vi "Teardown.vi"(8 "error in (no error)":errorcluster, 11 "LUnit Process Test In":refnum<class "Process Test.lvclass">) -> (0 "error out":errorcluster, 3 "LUnit Process Test Out":refnum<class "Process Test.lvclass">)   [LabVIEW 2020, in "Process Test.lvclass"]
uses:
  Process Test.lvclass
  Process Test.lvclass/Process Test.ctl
  C:/Git/astemes-triarc-framework/source/Framework Test Suite/Base Class Test/Base Test.lvclass
  C:/Program Files (x86)/National Instruments/LabVIEW 2020/vi.lib/Astemes/LUnit/Test Case.lvclass
  C:/Git/astemes-triarc-framework/source/Framework Test Suite/Process Test/Process Test.lvclass
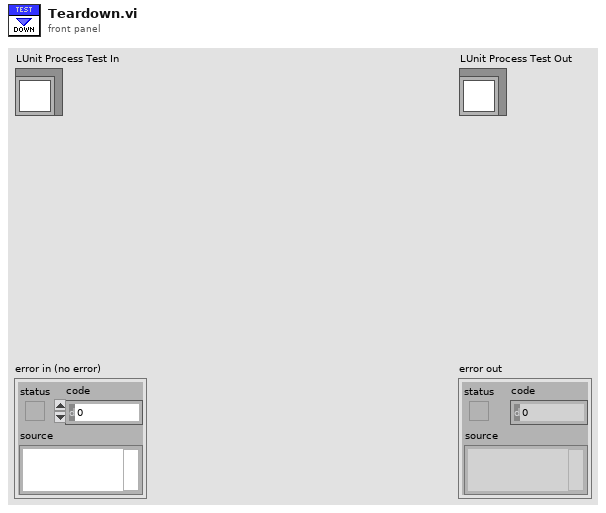
[diagram p1: front panel]
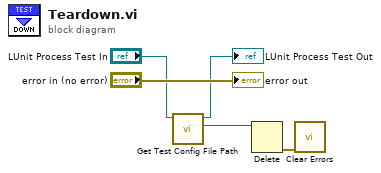
[diagram p0: block diagram]
diagram:
  n1 = call "Get Test Config File Path.vi"("Process Test In"="LUnit Process Test In") -> ("Test config path"=w3:path, "Process Test Out"=→"LUnit Process Test Out":refnum<class "Process Test.lvclass">)  [unwired: 8 in, 1 out]
  n2 = Delete(path (use dialog)=w3) -> (error out=w5:errorcluster)  [unwired: 4 in, 2 out]
  n3 = call <vilib>:"Clear Errors.vi"("error in (no error)"=w5) -> ()  [unwired: 5 in, 2 out]
  "error out" <- "error in (no error)"
